vi "MQTT Client - Disconnect.vi"(0 "MQTT Session":T1, 7 "With Will (v5)":bool=TRUE, 11 "error in (no error)":errorcluster) -> (4 "MQTT Session out":T1, 15 "error out":errorcluster)   [LabVIEW 2019, in "KoRE-MQTT.lvlib"]
doc: "<b>Description:</b> This VI gracefully disconnects from the MQTT broker. If a Will Message is configured for the session, this function will request the server to publish it. To ensure that the server only publishes the Will Message in the event of an unexpected disconnect, you must explicitly set Use Will to false.\n\nNotice: When a session is disconnected, all configured session settings—including username, password, and connection properties—are preserved. These settings will be automatically applied during subsequent reconnection attempts, unless they are explicitly reconfigured.\n\n<b>Input Terminals:</b>\n- <b>MQTT session [0]</b>: Reference to the MQTT session that will be disconnected.\n- <b>With Will (v5) [7]</b>: Boolean value indicating whether to publish a Will Message upon disconnection. Default value is false (MQTT v5 only).\n\n<b>Output Terminals:</b>\n- <b>error out [15]</b>: Error output that indicates the success or failure of the disconnect operation.\n\n\nCopyright (c) 2025 KoRElibs.com\nSPDX-License-Identifier: EUPL-1.2\n\nThis VI is licensed under the European Union Public License (EUPL) Version 1.2. You may use this VI unmodified in proprietary works. If you distribute a modified version of this file, the modified file must be released under the EUPL-1.2. Full license: https://joinup.ec.europa.eu/asset/eupl/eupl/1.2/"
uses:
  KoRE-MQTT.lvlib
  TypeDefs/MQTT Client Session.ctl
  Private/TypeDefs/MQTT Packet - Type.ctl
  Private/MQTT Session - Get TCP Info.vi
  Private/MQTT Session - Reset Keep Alive Timer.vi
  Private/MQTT Data Stream - Write Packet.vi
  Private/MQTT Data - Encode Varint.vi
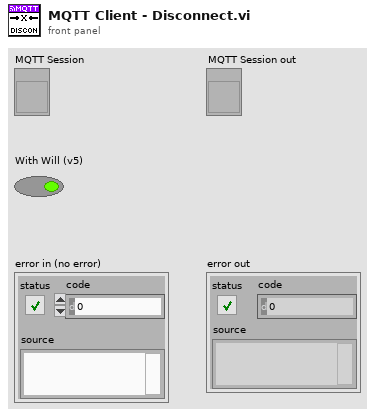
[diagram p1: front panel]
types:
  T1 = typedef "KoRE-MQTT.lvlib/MQTT Client Session.ctl" = refnum<vi>
  T2 = typedef "KoRE-MQTT.lvlib/MQTT Packet - Type.ctl" = enum32{"Reserved", "CONNECT", "CONNACK", "PUBLISH", "PUBACK", "PUBREC", "PUBREL", "PUBCOMP", "SUBSCRIBE", "SUBACK", "UNSUBSCRIBE", "UNSUBACK", "PINGREQ", "PINGRESP", "DISCONNECT", "AUTH"}
  T3 = typedef "KoRE-MQTT.lvlib/MQTT Client Session - Data.ctl" = cluster{"TCP ref":refnum<k5>, "Next Packet Id":u16, "Version":u8, "Host":string, "Port":u16, "Ping Delta":u32, "Username":string, "Password":string, "Will QoS":u8, "Will Retain":bool, "Will Topic":string, "Will Payload":string, "TCP Timeout":i32, "Semaphore":T4, "In-Flight Messages":variant, "Close":bool, "Last Send":u32, "Keep Alive":u16, "Last Ping RTT":u32, "Last Ping":u32, "Will Properties":T5[], "Session Expiry Interval":u32, "Maximum QoS":u8, "Retain Available":bool, "Server Maximum Packet Size":u32, "Client Identifier":string, "Server Topic Alias Maximum":u16, "Wildcard Subscription Available":bool, "Subscription Identifier Available":bool, "Shared Subscription Available":bool, "Connect Properties":T6[], "Client Maximum Packet Size":u32, "Client Topic Alias Maximum":u16, "Server Receive Maximum":u16, "Client Receive Maximum":u16, "TLS cfg":refnum<k36>, "Subscriptions":T7[]}
  T4 = typedef "Semaphore RefNum" = refnum<k1>
  T5 = typedef "KoRE-MQTT.lvlib/MQTT Property - Will.ctl" = cluster{"Property":u8, "Value":string}
  T6 = typedef "KoRE-MQTT.lvlib/MQTT Property - CONNECT.ctl" = cluster{"Property":u8, "Value":string}
  T7 = typedef "KoRE-MQTT.lvlib/MQTT Subscription - Info.ctl" = cluster{"Packet Id":u16, "Index":u16, "Identifier":u32, "QoS":u8, "Topic Filter":string, "Reason Code":u8, "Reason String":string, "Granted":bool}
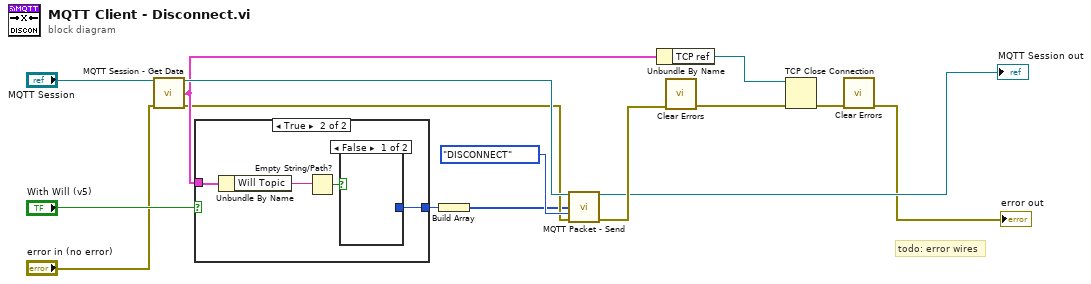
[diagram p0: block diagram]
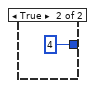
[diagram p3: hidden frame]
diagram:
  # "todo: error wires"
  n1 = call "MQTT Session - Get Data.vi"("mqtt ref in"="MQTT Session", "error in"="error in (no error)") -> ("mqtt ref out"=w12:T1, "mqtt ref data"=w11:T3, "error out"=w3:errorcluster)  [unwired: 11 in]
  n2 = case shown="True" "With Will (v5)" {
    tunnel: w11 -> [_ w19]
    tunnel: [_ w16] -> w9
    frame False {
    }
    frame True {
      n3 = Unbundle By Name(w19) -> ("Will Topic"=w18:string)
      n4 = Empty String/Path?(string/path=w18) -> (empty?=w17:bool)
      n5 = case shown="False" w17 {
        tunnel: [_ u8 4] -> w16
        frame False {
        }
        frame True {
        }
      }
    }
  }
  n6 = Build Array(w9) -> (w2:u8[])
  n7 = call "MQTT Packet - Send.vi"("mqtt ref in"=w12, "packet data"=w2, "MessageType"=MQTT_Packet_-_Type."DISCONNECT", "error in (no error)"=w3) -> ("mqtt ref out"=→"MQTT Session out":T1, "error out"=w5:errorcluster)  [unwired: 9 in, 1 out]
  n8 = Unbundle By Name(w11) -> ("TCP ref"=w13:refnum<k5>)
  n9 = call <vilib>:"Clear Errors.vi"("error in (no error)"=w5) -> ("error out"=w6:errorcluster)  [unwired: 5 in, 1 out]
  n10 = TCP Close Connection(connection ID=w13, error in (no error)=w6) -> (error out=w7:errorcluster)  [unwired: 1 in, 1 out]
  n11 = call <vilib>:"Clear Errors.vi"("error in (no error)"=w7) -> ("error out"=→"error out":errorcluster)  [unwired: 5 in, 1 out]
